vi "_CSMOFGV Dequeue.vi"(8 "Error In":errorcluster caption="error in (no error)", 9 "Dequeue Timeout (0ms)":i32, 10 "State (S) In (\"\")":string, 11 "CSMQ In":T1={"info"={"Module Name"="", "Requested Name"="", "Group Name"="", "Mode"=enum."Stand Alone", "Allowed Messages"=[]}, "Refs"={"WatchDogQ"=refnum, "CSMDataDVR"=refnum, "Queue"={"HPriorityQ"=refnum, "LowPriorityQ"=refnum}, "GroupDataDVR"=refnum, "TagMap"=refnum, "ExitEvent"=refnum, "NewStateEvent"=refnum, "StatusEvent"=refnum, "InterruptEvent"=refnum}}) -> (0 "error out":errorcluster, 2 "States Out":string, 3 "CSMQ Out":T1={"info"={"Module Name"="", "Requested Name"="", "Group Name"="", "Mode"=enum."Stand Alone", "Allowed Messages"=[]}, "Refs"={"WatchDogQ"=refnum, "CSMDataDVR"=refnum, "Queue"={"HPriorityQ"=refnum, "LowPriorityQ"=refnum}, "GroupDataDVR"=refnum, "TagMap"=refnum, "ExitEvent"=refnum, "NewStateEvent"=refnum, "StatusEvent"=refnum, "InterruptEvent"=refnum}})   [LabVIEW 2017, in "Communicable State Machine.lvlib"]
uses:
  Communicable State Machine.lvlib
  _CSMObj.ctl
  _CSMObj-Info.ctl
  Typedef/_CSM_MODE.ctl
  _CSMObj-Refs.ctl
  _CSMObj-Data.ctl
  Typedef/_CSM_MSG_TYPE.ctl
  Priority Queue/Priority Queue.ctl
  Typedef/_Cross CSM State Data.ctl
  Typedef/_Cross CSM State Response.ctl
  Typedef/_CSM_Response Source Message.ctl
  Priority Queue/def-Data(LowPRI-Q).ctl
  _CSMObj-ModeData.ctl
  Typedef/_CSM Status Change Event Data.ctl
  AdvanceAPI/CSM - Make String Arguments Safe.vi
  AdvanceAPI/CSM - Keywords.vi
  _Shared/CSM Shared.lvlib
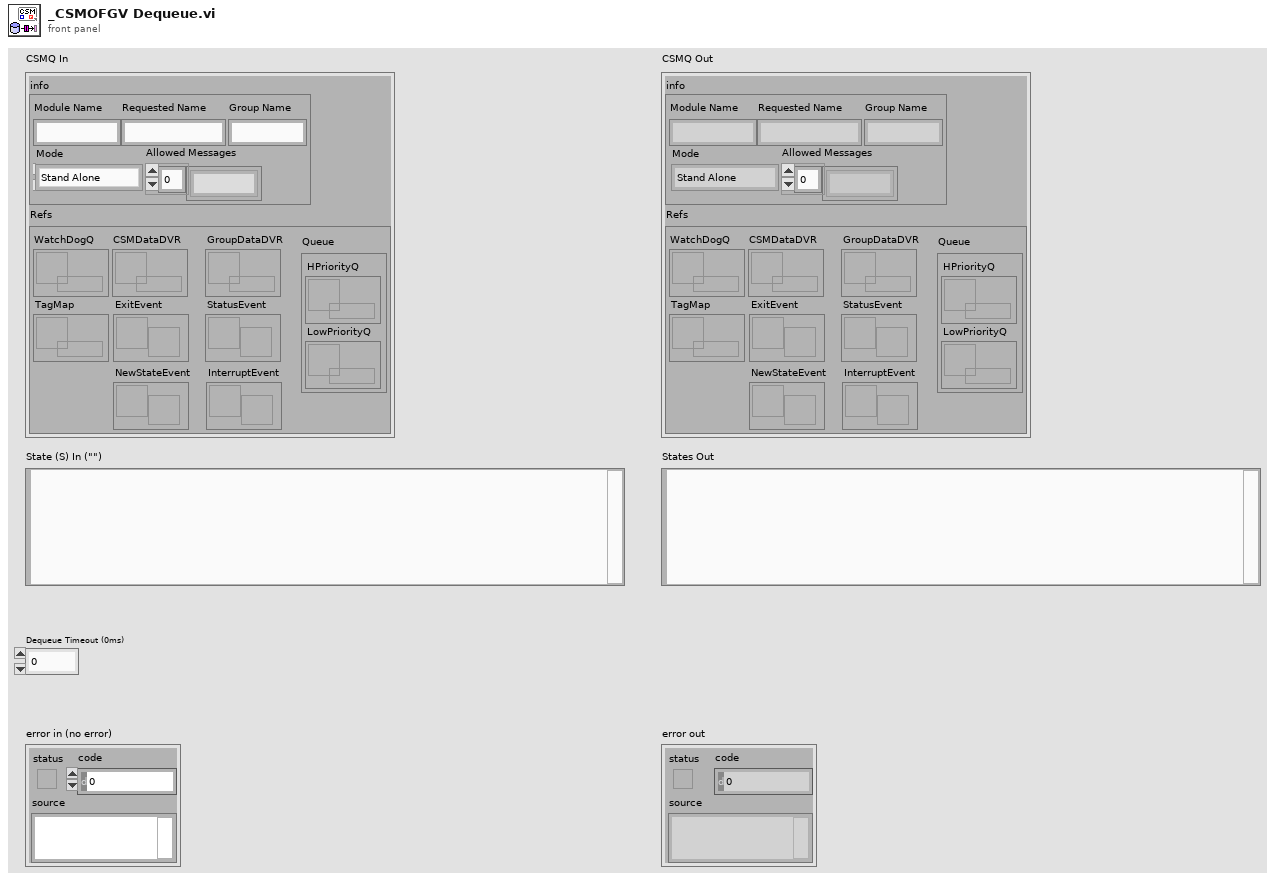
[diagram p1: front panel]
types:
  T1 = typedef "Communicable State Machine.lvlib/_CSMObj.ctl" = cluster{"info":T2, "Refs":T4}
  T2 = typedef "Communicable State Machine.lvlib/_CSMObj-Info.ctl" = cluster{"Module Name":string, "Requested Name":string, "Group Name":string, "Mode":T3, "Allowed Messages":string[]}
  T3 = typedef "Communicable State Machine.lvlib/_CSM_MODE.ctl" = enum16{"Not Exist", "Stand Alone", "CSM", "Worker", "Worker Agent", "Chain Node", "Chain"}
  T4 = typedef "Communicable State Machine.lvlib/_CSMObj-Refs.ctl" = cluster{"WatchDogQ":refnum<queue>, "CSMDataDVR":refnum<data-value>, "Queue":T5, "GroupDataDVR":refnum<data-value>, "TagMap":refnum<data-value>, "ExitEvent":refnum<user-event>, "NewStateEvent":refnum<user-event>, "StatusEvent":refnum<user-event>, "InterruptEvent":refnum<user-event>}
  T5 = typedef "Communicable State Machine.lvlib/Priority Queue.ctl" = cluster{"HPriorityQ":refnum<queue>, "LowPriorityQ":refnum<queue>}
  T6 = typedef "Communicable State Machine.lvlib/_CSM_MSG_TYPE.ctl" = enum16{"Sync Message(-@)", "Async Message(->)", "Async without Response(->|)", "Async Response", "Broadcast(-><all>)", "Broadcast(-><status>)", "Broadcast(-><interrupt>)", "Append to JKISM States", "Append to JKISM States(High Priority)", "Broadcast(-><state>)", "<None>"}
  T7 = typedef "Communicable State Machine.lvlib/_CSMObj-Data.ctl" = cluster{"RemoteMessge?":bool, "error":errorcluster, "Return State":string, "Initialized":enum16{"Initializing", "Ready", "Exiting"}, "InternalRegistryRules":string[], "Return Msg Type":T6, "Current State":string, "Remaing JKISM Queue":string}
  T8 = typedef "Communicable State Machine.lvlib/_Cross CSM State Data.ctl" = cluster{"Msg Type":T6, "state":string, "args":string, "source":string, "RespQ":refnum<queue>, "Response For Message":T9, "Target":string}
  T9 = typedef "Communicable State Machine.lvlib/_CSM_Response Source Message.ctl" = cluster{"‘State":string, "’Arguments":string, "’Error":errorcluster}
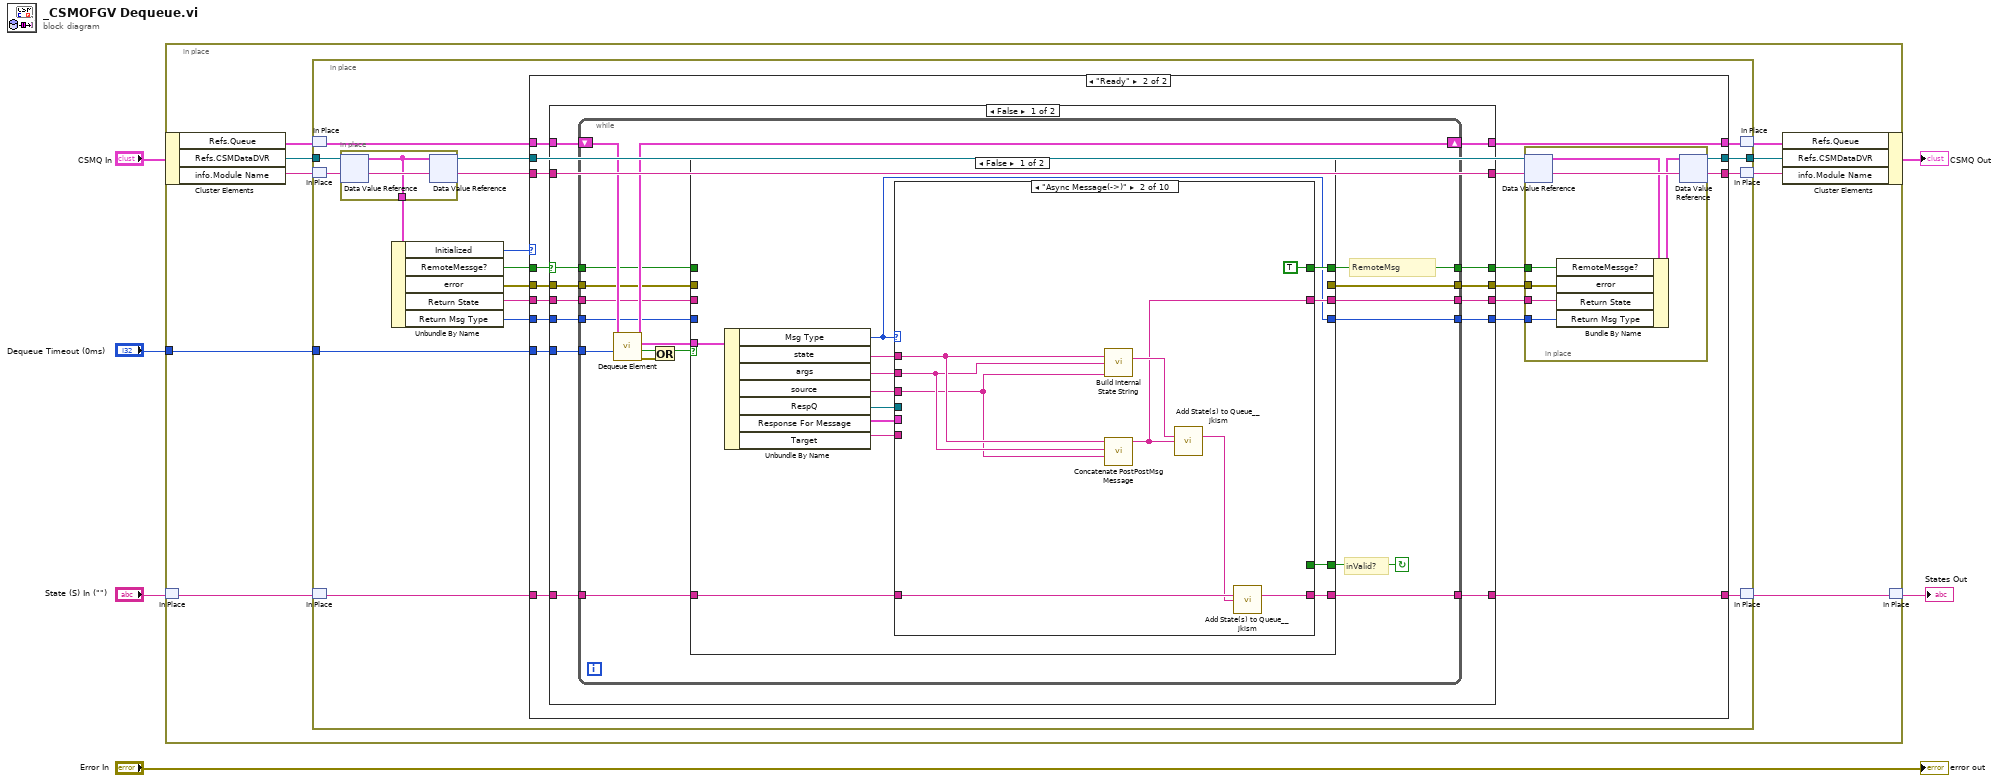
[diagram p0: block diagram]
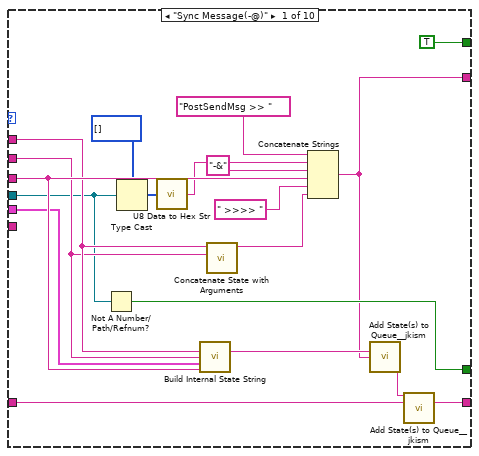
[diagram p3: hidden frame]
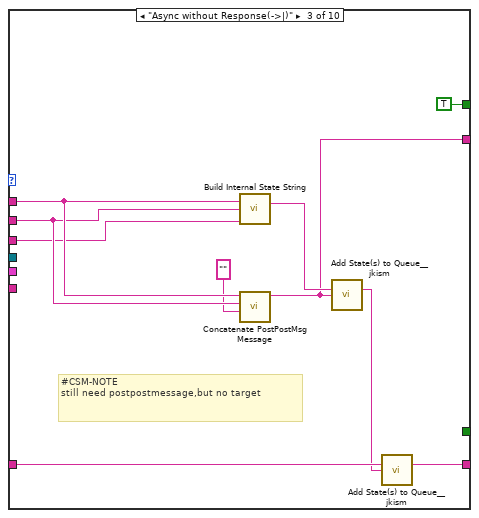
[diagram p4: hidden frame]
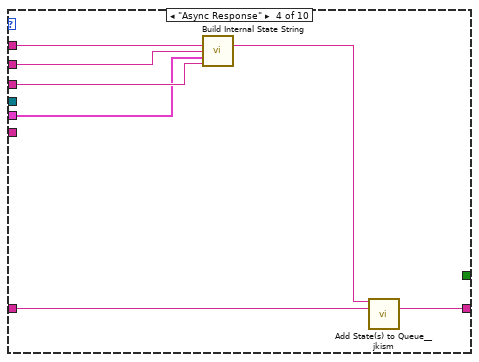
[diagram p5: hidden frame]
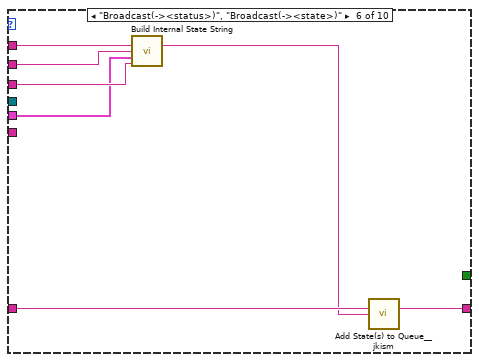
[diagram p7: hidden frame]
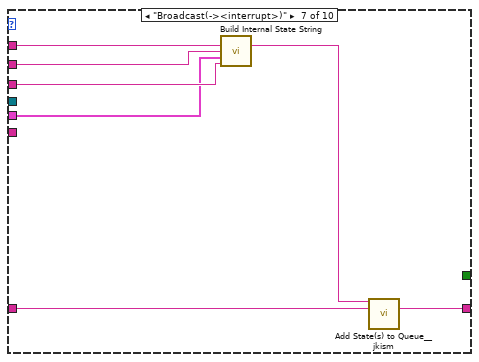
[diagram p8: hidden frame]
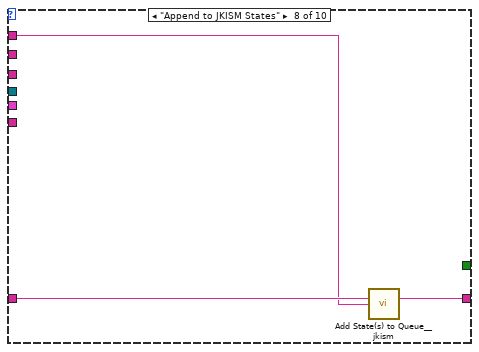
[diagram p9: hidden frame]
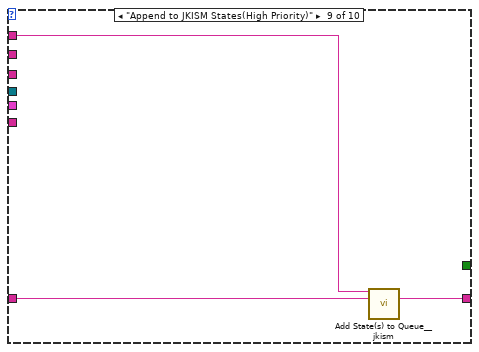
[diagram p10: hidden frame]
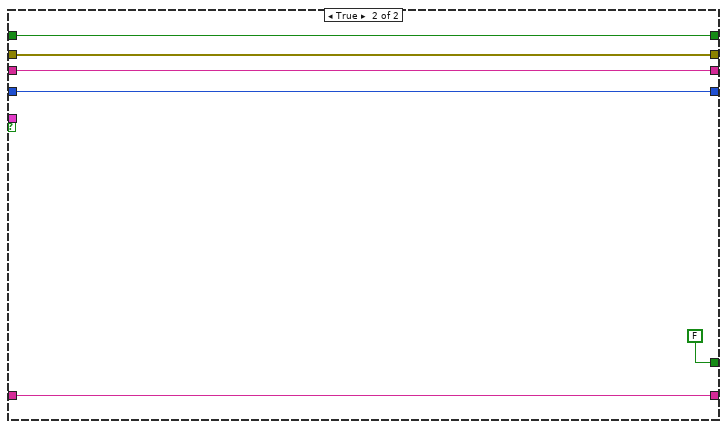
[diagram p12: hidden frame]
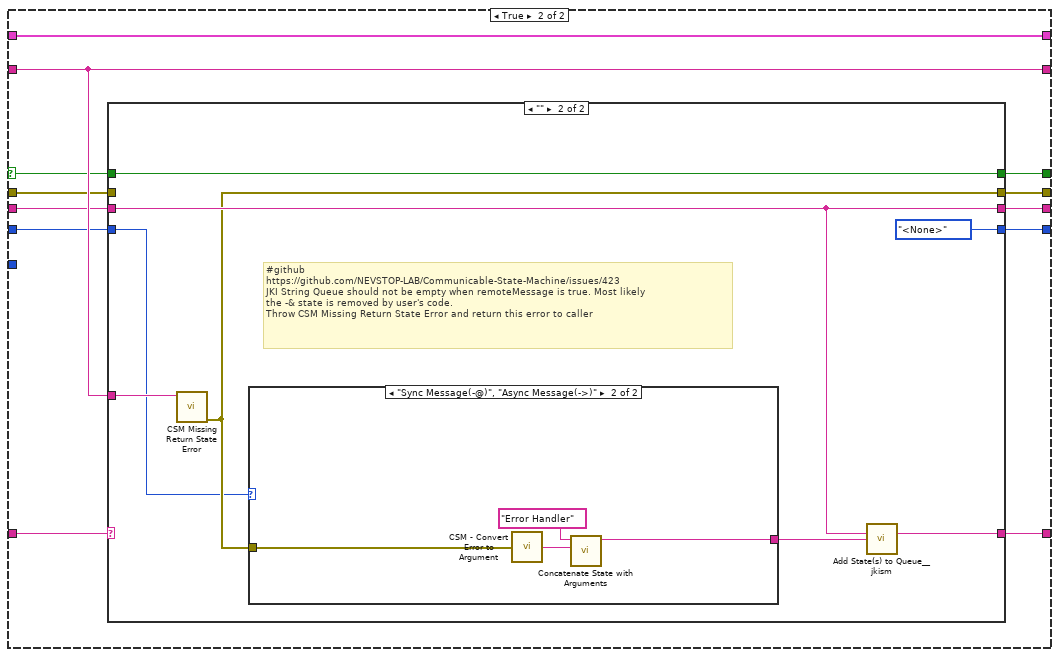
[diagram p13: hidden frame]
diagram:
  n1 = in-place "In Place Element Structure" {
    in-place-border: "Dequeue Timeout (0ms)" -> [w13]
    n2 = in-place-cluster #1("CSMQ In") -> ("Refs.Queue"=w15:T5, "Refs.CSMDataDVR"=w10:refnum<data-value>, "info.Module Name"=w7:string)
    n3 = in-place-match #2("State (S) In (\"\")") -> (w12:string)
    n4 = in-place {
      in-place-border: w13 -> [w29]
      in-place-border: w10 -> [w26]
      in-place-border: [w23] -> w9
      n5 = in-place-match #3(w15) -> (w30:T5)
      n6 = in-place-match #4(w7) -> (w19:string)
      n7 = in-place-match #5(w12) -> (w28:string)
      n8 = in-place {
        in-place-border: [w206] -> w25
        n9 = in-place-dvr #6(w26) -> (w206:T7)  [unwired: 1 out]
        n10 = in-place-dvr #6(w206) -> (w24:refnum<data-value>)  [unwired: 1 out]
      }
      n11 = Unbundle By Name(w25) -> ("Initialized"=w17:enum16{"Initializing", "Ready", "Exiting"}, "RemoteMessge?"=w22:bool, "error"=w21:errorcluster, "Return State"=w20:string, "Return Msg Type"=w16:T6)
      n12 = case shown="\"Ready\"" w17 {
        tunnel: [w35 w52] -> w31
        tunnel: w30 -> [w35 w51]
        tunnel: w29 -> [_ w50]
        tunnel: w28 -> [w32 w49]
        tunnel: [w32 w48] -> w27
        tunnel: w24 -> [w34 w47]
        tunnel: [w34 w46] -> w23
        tunnel: w22 -> [_ w44]
        tunnel: w21 -> [_ w42]
        tunnel: w20 -> [_ w40]
        tunnel: w19 -> [w33 w39]
        tunnel: [w33 w38] -> w18
        tunnel: w16 -> [_ w36]
        frame "Initializing", "Exiting", Default {
        }
        frame "Ready" {
          n13 = case shown="False" w44 {
            selector: w44 -> [w66 w179]
            tunnel: [w71 w188] -> w52
            tunnel: w51 -> [w72 w188]
            tunnel: w50 -> [w70 _]
            tunnel: w49 -> [w69 w182]
            tunnel: [w68 w181] -> w48
            tunnel: [w67 w180] -> w45
            tunnel: [w65 w186] -> w43
            tunnel: w42 -> [w64 w185]
            tunnel: [w63 w184] -> w41
            tunnel: w40 -> [w62 w183]
            tunnel: w39 -> [w61 w187]
            tunnel: [w61 w187] -> w38
            tunnel: [w60 w178] -> w37
            tunnel: w36 -> [w59 w177]
            frame False {
              n14 = while {
                tunnel: w70 -> [w88]
                shift-right: [w89] -> w71
                shift-left: w72 -> [w90]
                tunnel: w66 -> [w80]
                tunnel: [w81] -> w67
                tunnel: w69 -> [w86]
                tunnel: [w85] -> w68
                tunnel: [w78] -> w65
                tunnel: w64 -> [w77]
                tunnel: [w76] -> w63
                tunnel: w62 -> [w75]
                tunnel: [w74] -> w60
                tunnel: w59 -> [w73]
                stop <- w79 continue-if-true
                # "inValid?"
                # "RemoteMsg"
                n15 = call "Dequeue Element.vi"("Timeout In ms (-1)"=w88, "Priority Queue"=w90) -> ("error out"=w82:errorcluster, "Timed Out?"=w83:bool, "Cross JKI State Machine State"=w87:T8, "Priority Queue (Dup)"=w89:T5)  [unwired: 5 in, 1 out]
                n16 = Or(x=w83, y=w82) -> (x .or. y?=w84:bool)
                n17 = case shown="False" w84 {
                  tunnel: w86 -> [w103 w176]
                  tunnel: [w102 w176] -> w85
                  tunnel: w87 -> [w97 _]
                  tunnel: [w94 w175] -> w81
                  tunnel: w80 -> [_ w175]
                  tunnel: [w93 FALSE] -> w79
                  tunnel: [_ w173] -> w78
                  tunnel: w77 -> [_ w173]
                  tunnel: [w92 w172] -> w76
                  tunnel: w75 -> [_ w172]
                  tunnel: [w91 w171] -> w74
                  tunnel: w73 -> [_ w171]
                  frame False {
                    n18 = Unbundle By Name(w97) -> ("Msg Type"=w91:T6, "state"=w100:string, "args"=w99:string, "source"=w98:string, "RespQ"=w101:refnum<queue>, "Response For Message"=w96:T9, "Target"=w95:string)
                    n19 = case shown="\"Async Message(->)\"" w91 {
                      tunnel: w103 -> [w122 w131 w141 w148 w149 w156 w163 w166 w169 w170]
                      tunnel: [w121 w130 w140 w147 w149 w155 w162 w165 w168 w170] -> w102
                      tunnel: w101 -> [w106 _ _ _ _ _ _ _ _ _]
                      tunnel: w100 -> [w112 w126 w136 w144 _ w152 w159 w164 w167 _]
                      tunnel: w99 -> [w111 w125 w135 w146 _ w154 w161 _ _ _]
                      tunnel: w98 -> [w115 w124 w134 w145 _ w153 w160 _ _ _]
                      tunnel: w96 -> [w113 _ _ w142 _ w151 w158 _ _ _]
                      tunnel: w95 -> [_ _ _ _ _ _ _ _ _ _]
                      tunnel: [TRUE TRUE TRUE _ _ _ _ _ _ _] -> w94
                      tunnel: [w105 _ _ _ _ _ _ _ _ _] -> w93
                      tunnel: [w104 w123 w132 _ _ _ _ _ _ _] -> w92
                      frame "Sync Message(-@)" {
                        n20 = Not A Number/Path/Refnum?(number/path/refnum=w106) -> (NaN/Path/Refnum?=w105:bool)
                        n21 = Type Cast(type=u8[] [], x=w106) -> (*(type *) &x=w108:u8[])
                        n22 = call "U8 Data to Hex Str.vi"("U8 Data[]"=w108) -> ("HEX String (0-9,A-F)"=w107:string)
                        n23 = call "Build Internal State String.vi"("State"=w112, "Arguments (\"\")"=w111, "Additional Information"=w113, "Source (\"\")"=w115) -> ("State With Arguments"=w118:string)  [unwired: 11 in]
                        n24 = call "Concatenate State with Arguments.vi"("Arguments"=w111, "State"=w112) -> ("State With Arguements"=w110:string)  [unwired: 9 in]
                        n25 = Concatenate Strings("PostSendMsg >> " ("State(s) at Back (\"\")"), w107, "-&" ("string"), w115, " >>>> " ("string"), w110) -> (w104:string)
                        n26 = call "Add State(s) to Queue__jkism.vi"("State(s) in (\"\")"=w118, "State(s) at Back (\"\")"=w104) -> ("States Out"=w120:string)  [unwired: 13 in]
                        n27 = call "Add State(s) to Queue__jkism.vi"("State(s) in Front (\"\")"=w120, "State(s) in (\"\")"=w122) -> ("States Out"=w121:string)  [unwired: 13 in]
                      }
                      frame "Async Message(->)" {
                        n28 = call "Build Internal State String.vi"("State"=w126, "Arguments (\"\")"=w125, "Source (\"\")"=w124) -> ("State With Arguments"=w129:string)  [unwired: 12 in]
                        n29 = call "Concatenate PostPostMsg Message.vi"("Source"=w124, "Arguments"=w125, "Async-Message"=w126) -> ("PostPostMsg Message"=w123:string)  [unwired: 8 in]
                        n30 = call "Add State(s) to Queue__jkism.vi"("State(s) in (\"\")"=w129, "State(s) at Back (\"\")"=w123) -> ("States Out"=w127:string)  [unwired: 13 in]
                        n31 = call "Add State(s) to Queue__jkism.vi"("State(s) in (\"\")"=w131, "State(s) at Back (\"\")"=w127) -> ("States Out"=w130:string)  [unwired: 13 in]
                      }
                      frame "Async without Response(->|)" {
                        # "#CSM-NOTE\nstill need postpostmessage,but no target"
                        n32 = call "Build Internal State String.vi"("State"=w136, "Arguments (\"\")"=w135, "Source (\"\")"=w134) -> ("State With Arguments"=w139:string)  [unwired: 12 in]
                        n33 = call "Concatenate PostPostMsg Message.vi"("Source"="", "Arguments"=w135, "Async-Message"=w136) -> ("PostPostMsg Message"=w132:string)  [unwired: 8 in]
                        n34 = call "Add State(s) to Queue__jkism.vi"("State(s) in (\"\")"=w139, "State(s) at Back (\"\")"=w132) -> ("States Out"=w137:string)  [unwired: 13 in]
                        n35 = call "Add State(s) to Queue__jkism.vi"("State(s) in (\"\")"=w141, "State(s) at Back (\"\")"=w137) -> ("States Out"=w140:string)  [unwired: 13 in]
                      }
                      frame "Async Response" {
                        n36 = call "Build Internal State String.vi"("State"=w144, "Arguments (\"\")"=w146, "Additional Information"=w142, "Source (\"\")"=w145) -> ("State With Arguments"=w143:string)  [unwired: 11 in]
                        n37 = call "Add State(s) to Queue__jkism.vi"("State(s) in Front (\"\")"=w143, "State(s) in (\"\")"=w148) -> ("States Out"=w147:string)  [unwired: 13 in]
                      }
                      frame "Broadcast(-><all>)" {
                        # "#CSM-NOTE\nshould no be here"
                      }
                      frame "Broadcast(-><status>)", "Broadcast(-><state>)" {
                        n38 = call "Build Internal State String.vi"("State"=w152, "Arguments (\"\")"=w154, "Additional Information"=w151, "Source (\"\")"=w153) -> ("State With Arguments"=w150:string)  [unwired: 11 in]
                        n39 = call "Add State(s) to Queue__jkism.vi"("State(s) in (\"\")"=w156, "State(s) at Back (\"\")"=w150) -> ("States Out"=w155:string)  [unwired: 13 in]
                      }
                      frame "Broadcast(-><interrupt>)" {
                        n40 = call "Build Internal State String.vi"("State"=w159, "Arguments (\"\")"=w161, "Additional Information"=w158, "Source (\"\")"=w160) -> ("State With Arguments"=w157:string)  [unwired: 11 in]
                        n41 = call "Add State(s) to Queue__jkism.vi"("State(s) in Front (\"\")"=w157, "State(s) in (\"\")"=w163) -> ("States Out"=w162:string)  [unwired: 13 in]
                      }
                      frame "Append to JKISM States" {
                        n42 = call "Add State(s) to Queue__jkism.vi"("State(s) in (\"\")"=w166, "State(s) at Back (\"\")"=w164) -> ("States Out"=w165:string)  [unwired: 13 in]
                      }
                      frame "Append to JKISM States(High Priority)" {
                        n43 = call "Add State(s) to Queue__jkism.vi"("State(s) in Front (\"\")"=w167, "State(s) in (\"\")"=w169) -> ("States Out"=w168:string)  [unwired: 13 in]
                      }
                      frame "<None>" {
                      }
                    }
                  }
                  frame True {
                  }
                }
              }
            }
            frame True {
              n44 = case shown="\"\"" w182 {
                selector: w182 -> [w191 _]
                tunnel: w187 -> [_ w201]
                tunnel: [w193 w198] -> w186
                tunnel: w185 -> [w193 _]
                tunnel: [w192 w199] -> w184
                tunnel: w183 -> [w192 w199]
                tunnel: [w191 w200] -> w181
                tunnel: [w190 w195] -> w180
                tunnel: w179 -> [w190 w195]
                tunnel: [w189 _CSM_MSG_TYPE."<None>" ("Return Msg Type")] -> w178
                tunnel: w177 -> [w189 w194]
                frame Default {
                }
                frame "" {
                  # "#github \nhttps://github.com/NEVSTOP-LAB/Communicable-State-Machine/issues/423\nJKI String Queue should not be empty when remoteMessage is true. Most likely\nthe -& state is removed by user's code. \nThrow CSM Missing Return State Error and return this error to caller"
                  n45 = call "CSM Missing Return State Error.vi"("Arguments (As CSM Name)"=w201) -> ("error out"=w198:errorcluster)  [unwired: 10 in]
                  n46 = case shown="\"Sync Message(-@)\", \"Async Message(->)\"" w194 {
                    tunnel: w198 -> [_ w205]
                    tunnel: [_ w204] -> w196
                    frame "Async without Response(->|)", Default {
                    }
                    frame "Sync Message(-@)", "Async Message(->)" {
                      n47 = call "CSM - Convert Error to Argument.vi"("Error"=w205) -> ("Argument"=w203:string)  [unwired: 4 in]
                      n48 = call "Concatenate State with Arguments.vi"("Arguments"=w203, "State"="Error Handler") -> ("State With Arguements"=w204:string)  [unwired: 9 in]
                    }
                  }
                  n49 = call "Add State(s) to Queue__jkism.vi"("State(s) in (\"\")"=w199, "State(s) at Back (\"\")"=w196) -> ("States Out"=w200:string)  [unwired: 13 in]
                }
              }
            }
          }
          n50 = in-place {
            in-place-border: w45 -> [w56]
            in-place-border: w43 -> [w55]
            in-place-border: w41 -> [w54]
            in-place-border: w37 -> [w53]
            n51 = in-place-dvr #7(w47) -> (w58:T7)  [unwired: 1 out]
            n52 = Bundle By Name(cluster=w58, "RemoteMessge?"=w56, "error"=w55, "Return State"=w54, "Return Msg Type"=w53) -> (w57:T7)
            n53 = in-place-dvr #7(w57) -> (w46:refnum<data-value>)  [unwired: 1 out]
          }
        }
      }
      n54 = in-place-match #3(w31) -> (w14:T5)
      n55 = in-place-match #4(w18) -> (w8:string)
      n56 = in-place-match #5(w27) -> (w11:string)
    }
    n57 = in-place-cluster #1("Refs.Queue"=w14, "Refs.CSMDataDVR"=w9, "info.Module Name"=w8) -> (→"CSMQ Out":T1)
    n58 = in-place-match #2(w11) -> (→"States Out":string)
  }
  "error out" <- "Error In"
